vi "mupGetExpr.vi"(8 "error in (no error)":errorcluster, 11 "muPar in":u64) -> (0 "error out":errorcluster, 2 "expr":string, 3 "muPar out":u64)   [LabVIEW 2018, in "mupLib.lvlib"]
doc: "Get the expression string"
uses:
  mupLib.lvlib
  libmuparser-lv.dll
panel:
  # "Get the expression string"
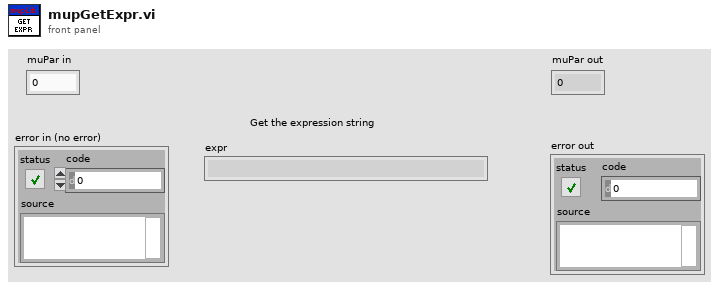
[diagram p1: front panel]
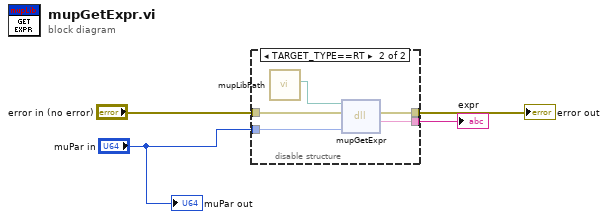
[diagram p0: block diagram]
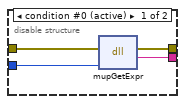
[diagram p2: hidden frame]
diagram:
  n1 = disable-structure shown="TARGET_TYPE==RT" {
    disable-tunnel: [w8 w13] -> w4
    disable-tunnel: "error in (no error)" -> [w7 w12]
    disable-tunnel: [w6 w11] -> w2
    disable-tunnel: "muPar in" -> [w5 w10]
    frame condition #0 (active) {
      n2 = dll-call lib="C:/Users/leonidas/Documents/GitHub/LV-muParser/mupLib/libmuparser-lv.dll" fn="mupGetExpr"(error in=w7, "hParser"=w5) -> (error out=w6:errorcluster, "expr"=w8:string)  [unwired: 3 in, 1 out]
    }
    frame condition #1 {
      n3 = call "mupLibPath.vi"() -> ("libmuparser path"=w9:path)  [unwired: 11 in]
      n4 = dll-call lib="C:/Users/leonidas/Documents/GitHub/LV-muParser/mupLib/libmuparser-lv.dll" fn="mupGetExpr"(path in=w9, error in=w12, "hParser"=w10) -> (error out=w11:errorcluster, "expr"=w13:string)  [unwired: 2 in, 1 out]
    }
  }
  "error out" <- w2
  "expr" <- w4
  "muPar out" <- "muPar in"
